vi "Serial_test.vi"() -> ()   [LabVIEW 2026]
panel:
  out "Reply":string
  in  "ESP32_Data":refnum<visa-resource-name>="COM20"
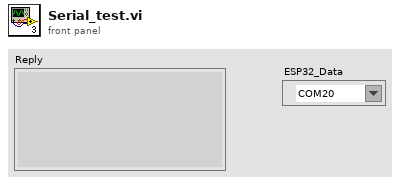
[diagram p1: front panel]
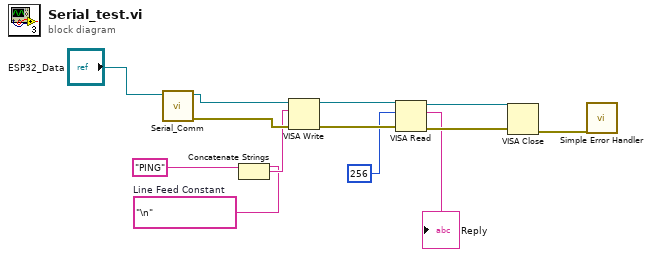
[diagram p0: block diagram]
diagram:
  w3 = "\n"  # Line Feed Constant
  n1 = call "Serial_Comm.vi"("ESP32_Data"="ESP32_Data") -> ("Roll_result"=w11:refnum<visa-resource-name>, "error out"=w8:errorcluster)  [unwired: 8 in]
  n2 = Concatenate Strings("PING", w3) -> (w5:string)
  n3 = VISA Write(VISA resource name=w11, write buffer=w5, error in (no error)=w8) -> (VISA resource name out=w10:refnum<visa-resource-name>, error out=w7:errorcluster)  [unwired: 1 out]
  n4 = VISA Read(VISA resource name=w10, byte count=u32 256, error in (no error)=w7) -> (VISA resource name out=w9:refnum<visa-resource-name>, read buffer=→"Reply":string, error out=w6:errorcluster)  [unwired: 1 out]
  n5 = VISA Close(VISA resource name=w9, error in (no error)=w6) -> (error out=w12:errorcluster)
  n6 = call <vilib>:"Simple Error Handler.vi"("error in (no error)"=w12) -> ()  [unwired: 4 in, 5 out]
